vi "Initialise.vi"(8 "error in (no error)":errorcluster, 11 "Dependency":variant) -> (0 "error out":errorcluster, 3 "Provider out":refnum<class "Provider.lvclass">)   [LabVIEW 2024, in "Provider.lvclass"]
uses:
  Provider.lvclass
  Provider.lvclass/Provider.ctl
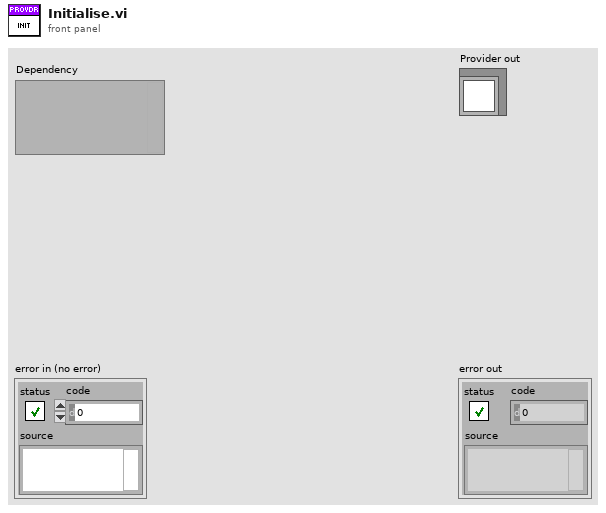
[diagram p1: front panel]
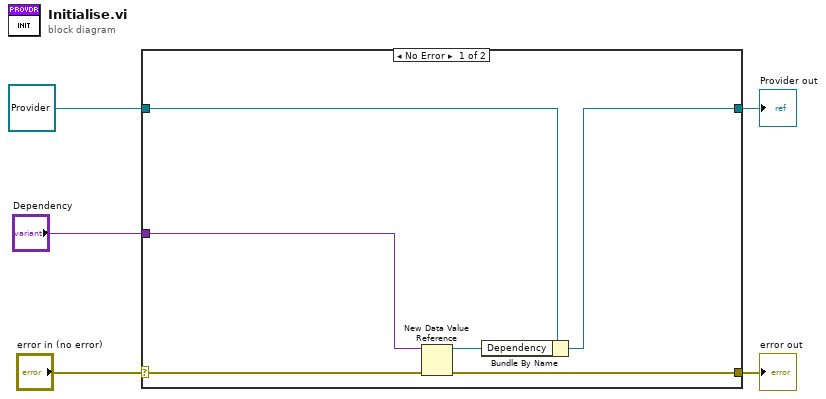
[diagram p0: block diagram]
diagram:
  n1 = case shown="No Error" "error in (no error)" {
    selector: "error in (no error)" -> [w10 w13]
    tunnel: [w9 w13] -> w4
    tunnel: [w6 w12] -> w2
    tunnel: refnum<class "Provider.lvclass"> refnum ("Provider in") -> [w8 w12]
    tunnel: "Dependency" -> [w11 _]
    frame No Error {
      n2 = New Data Value Reference(data value=w11, error in=w10) -> (data value reference=w7:refnum<data-value>, error out=w9:errorcluster)
      n3 = Bundle By Name(cluster=w8, "Dependency"=w7) -> (w6:refnum<class "Provider.lvclass">)
    }
    frame Error {
    }
  }
  "error out" <- w4
  "Provider out" <- w2
